vi "Get Start Impedence.vi"(8 "error in (no error)":errorcluster caption="错误输入（无错误）", 9 "nImpedence":u32, 10 "nBoard":i32, 11 "nDevId":i32) -> (0 "error out":errorcluster caption="错误输出", 1 "nImpedence out":u32, 3 "function return":i32)   [LabVIEW 2017, in "smncsftmt.lvlib"]
doc: "__declspec(dllexport) int GetStartImpedence(int nDevId, int nBoard, unsigned int* nImpedence);"
uses:
  smncsftmt.lvlib
  smncsftmt.dll
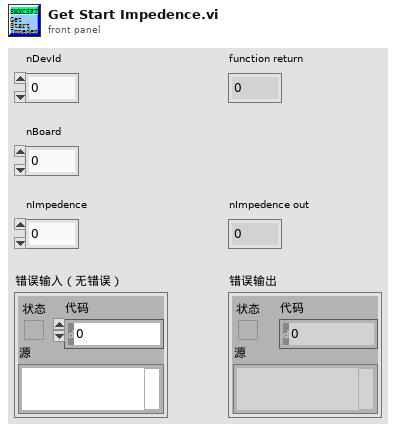
[diagram p1: front panel]
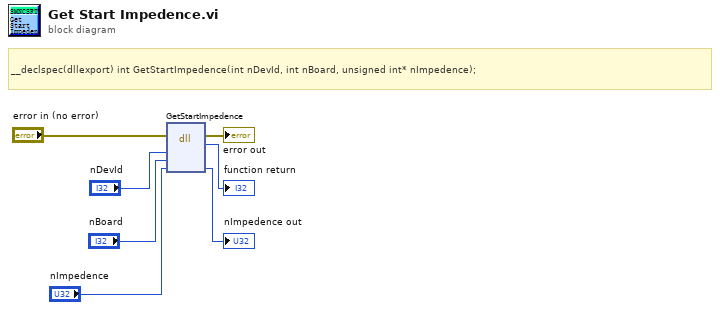
[diagram p0: block diagram]
diagram:
  # "__declspec(dllexport) int GetStartImpedence(int nDevId, int nBoard, unsigned int* nImpedence);"
  n1 = dll-call lib="PTH2oabs CUsersaDesktop\nLABVIEW范例National InstrumentsLabVIEW 2017user.lib\tsmncsftmtsmncsftmt.*" fn="GetStartImpedence"(error in="error in (no error)", "nDevId"="nDevId", "nBoard"="nBoard", "nImpedence"="nImpedence") -> (error out=→"error out":errorcluster, →"function return":i32, "nImpedence"=→"nImpedence out":u32)  [unwired: 4 in, 1 out]
